vi "Semaphore Name.vi"() -> (3 "semaphore name":string)   [LabVIEW 2018, in "GLog.lvlib" / "Registry.lvlib"]
uses:
  Registry.lvlib
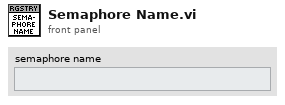
[diagram p1: front panel]
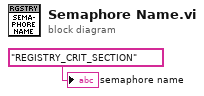
[diagram p0: block diagram]
diagram:
  "semaphore name" <- "REGISTRY_CRIT_SECTION" ("name (unnamed)")
